vi "Measure.vi"(8 "error in (no error)":errorcluster, 9 "measurement configuration":variant, 10 "measure call context in":refnum<class "Measure Call Context.lvclass">, 11 "measurement plugin in":refnum<class "Digital Pattern Sequencer.lvclass">) -> (0 "error out":errorcluster, 1 "measurement results":variant, 2 "measure call context out":refnum<class "Measure Call Context.lvclass">, 3 "measurement plugin out":refnum<class "Digital Pattern Sequencer.lvclass">)   [LabVIEW 2025, in "Digital Pattern Sequencer.lvclass"]
uses:
  Digital Pattern Sequencer.lvclass
  <vilib>/Plug-In SDKs/Measurements/Measure Call Context/Measure Call Context.lvclass
  Measurement Configuration.ctl
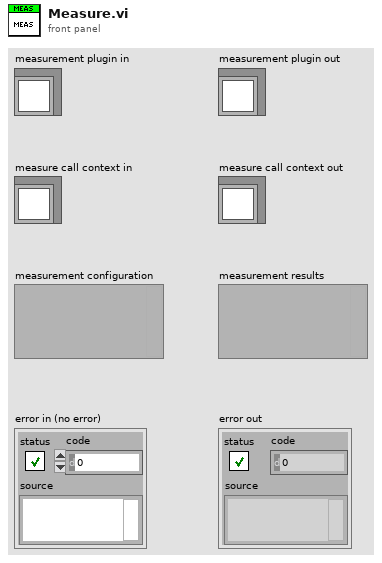
[diagram p1: front panel]
types:
  T1 = typedef "Digital Pattern Sequencer.lvclass/Measurement Configuration.ctl" = cluster{"DPE Project File Path":string, "Site":i32, "DUT Bring Up":string, "Apply TDR?":bool, "List-Patterns":string[], "List-Current Measurement Pins":string[]}
  T2 = typedef "Digital Pattern Sequencer.lvclass/Measurement Results.ctl" = cluster{"All Pass?":bool, "Results":string}
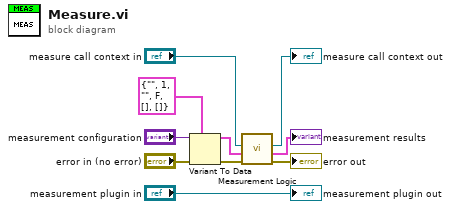
[diagram p0: block diagram]
diagram:
  n1 = Variant To Data(error in="error in (no error)", type=T1 {"DPE Project File Path"="", "Site"=1, "DUT Bring Up"="", "Apply TDR?"=FALSE, "List-Patterns"=[], "List-Current Measurement Pins"=[]} ("measurement configuration"), Variant="measurement configuration") -> (data=w1:T1, error out=w7:errorcluster)
  n2 = call "Measurement Logic.vi"("error in"=w7, "measurement configuration"=w1, "measure call context in"="measure call context in") -> ("error out"=→"error out":errorcluster, "measurement results"=→"measurement results":T2, "measure call context out"=→"measure call context out":refnum<class "Measure Call Context.lvclass">)  [unwired: 6 in]
  "measurement plugin out" <- "measurement plugin in"
